vi "MouseLUT.vi"(5 "axis info":T1, 7 "button info":T2, 8 "error in (no error)":errorcluster, 9 "Keyboard Key Pressed":T4(ring), 10 "Sample Number":u32, 11 "LUT Selector":T3) -> (0 "error out":errorcluster, 2 "axis info out":T1, 3 "button info out":T2)   [LabVIEW 2026, in "Core.lvlib"]
uses:
  modules/coordinator/src/Libraries/Core/Core.lvlib
  modules/coordinator/src/Libraries/MouseLUTSelector.ctl
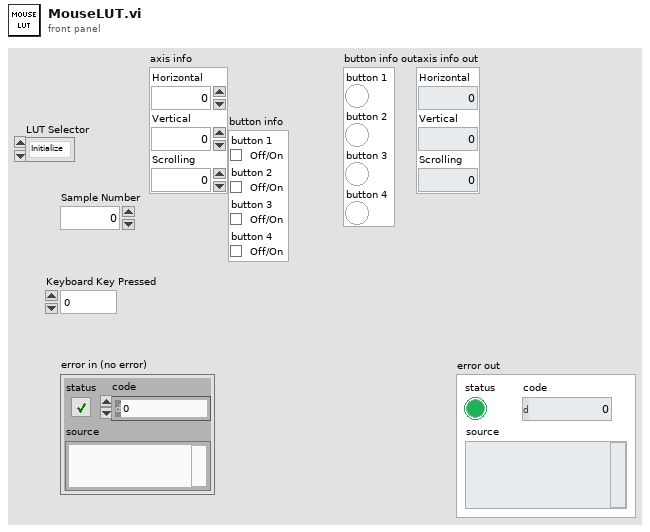
[diagram p1: front panel]
types:
  T1 = cluster{"Horizontal":i32, "Vertical":i32, "Scrolling":i32}
  T2 = cluster{"button 1":bool, "button 2":bool, "button 3":bool, "button 4":bool}
  T3 = typedef "Core.lvlib/MouseLUTSelector.ctl" = enum16{"Initialize", "Get Button and Axis Info", "Assign Button and Axis Info to Sample Number"}
  T4 = enum16{"0", "1", "2", "3", "4", "5", "6", "7", "8", "9", "A", "B", "C", "D", "E", "F", "G", "H", "I", "J", "K", "L", "M", "N", "O", "P", "Q", "R", "S", "T", "U", "V", "W", "X", "Y", "Z", "F1", "F2", "F3", "F4", "F5", "F6", "F7", "F8", "F9", "F10", "F11", "F12", "F13", "F14", "F15", "ADD", "BACK", "BACKSLASH", "CAPITAL", "COMMA", "DECIMAL", "DELETE", "DIVIDE", "DOWN", "END", "EQUALS", "ESCAPE", "GRAVE (`)", "HOME", "INSERT", "LBRACKET", "LCONTROL", "LEFT", "L ALT", "LSHIFT", "LWIN", "MINUS", "MULTIPLY", "NEXT", "NUMLOCK", "NUMPAD_0", "NUMPAD_1", "NUMPAD_2", "NUMPAD_3", "NUMPAD_4", "NUMPAD_5", "NUMPAD_6", "NUMPAD_7", "NUMPAD_8", "NUMPAD_9", "PAUSE", "PERIOD", "PRIOR (PG UP)", "RBRACKET", "RCONTROL", "RETURN", "RIGHT", "R ALT", "RSHIFT", "RWIN", "SCROLL", "SEMICOLON", "SLASH", "SPACE", "SUBTRACT", "TAB", "UP", "ENTER (num pad)", "' (quote)"}
  T5 = cluster{"button info":cluster{"button 1":bool, "button 2":bool, "button 3":bool, "button 4":bool}, "axis info":cluster{"Horizontal":i32, "Vertical":i32, "Scrolling":i32}}
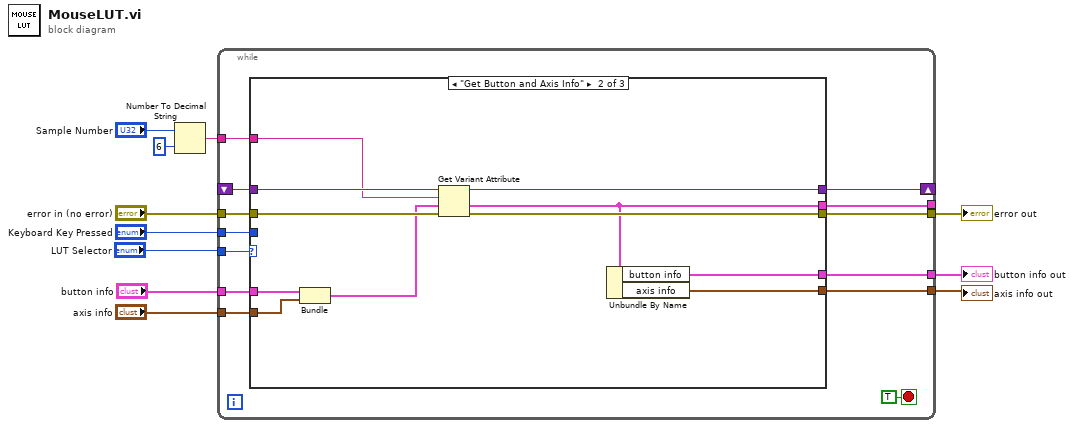
[diagram p0: block diagram]
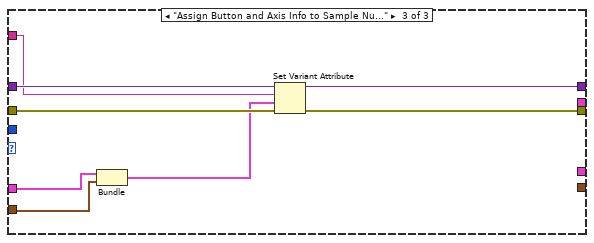
[diagram p3: hidden frame]
diagram:
  n1 = Number To Decimal String(number="Sample Number", width (-)=i16 6) -> (decimal integer string=w7:string)
  n2 = while {
    tunnel: "LUT Selector" -> [w23]
    shift-right: [w22] -> _
    shift-left: _ -> [w21]
    tunnel: w7 -> [w20]
    tunnel: [w19] -> w11
    tunnel: "Keyboard Key Pressed" -> [w18]
    tunnel: [w17] -> _
    tunnel: "error in (no error)" -> [w16]
    tunnel: "button info" -> [w15]
    tunnel: "axis info" -> [w14]
    tunnel: [w13] -> w2
    tunnel: [w12] -> w1
    stop <- TRUE stop-if-true
    n3 = case shown="\"Get Button and Axis Info\"" w23 {
      tunnel: [variant w36 w44] -> w22
      tunnel: w21 -> [_ w37 w45]
      tunnel: w20 -> [_ w34 w42]
      tunnel: [w25 w35 w43] -> w19
      tunnel: w18 -> [_ _ _]
      tunnel: [_ w29 _] -> w17
      tunnel: w16 -> [w25 w33 w41]
      tunnel: w15 -> [_ w32 w40]
      tunnel: w14 -> [_ w31 w39]
      tunnel: [_ w28 _] -> w13
      tunnel: [_ w27 _] -> w12
      frame "Initialize", Default {
      }
      frame "Get Button and Axis Info" {
        n4 = Bundle("button info"=w32, "axis info"=w31) -> (w30:T5)  [unwired: 1 in]
        n5 = Get Variant Attribute(Variant=w37, name=w34, default value (empty Variant)=w30, error in=w33) -> (duplicate Variant=w36:variant, value=w29:T5, error out=w35:errorcluster)  [unwired: 1 out]
        n6 = Unbundle By Name(w29) -> ("button info"=w28:T2, "axis info"=w27:T1)
      }
      frame "Assign Button and Axis Info to Sample Number" {
        n7 = Bundle("button info"=w40, "axis info"=w39) -> (w38:T5)  [unwired: 1 in]
        n8 = Set Variant Attribute(Variant=w45, name=w42, value=w38, error in=w41) -> (Variant out=w44:variant, error out=w43:errorcluster)  [unwired: 1 out]
      }
    }
  }
  "error out" <- w11
  "button info out" <- w2
  "axis info out" <- w1
